vi "MDPtr GlobalSettings.vi"(6 "Oper(Get)":bool, 8 "error in (no error)":errorcluster, 11 "Setting in":T1) -> (0 "error out":errorcluster, 3 "Setting out":T1)   [LabVIEW 2017, in "MDPtr.lvlib"]
uses:
  MDPtr.lvlib
  MDPtr TypeDef/MDPtr GlobalSettings.ctl
  MDPtr TypeDef/MDPtr MallocMethod.ctl
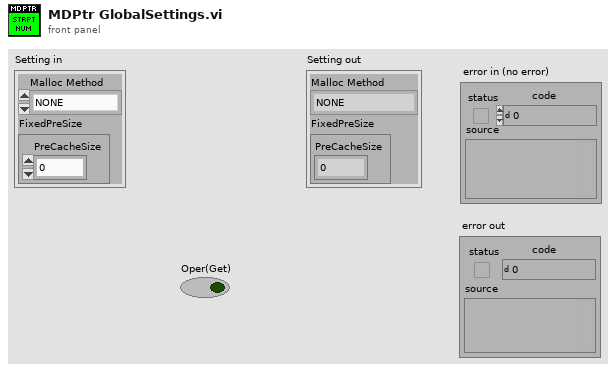
[diagram p1: front panel]
types:
  T1 = typedef "MDPtr.lvlib/MDPtr GlobalSettings.ctl" = cluster{"Malloc Method":T2, "FixedPreSize":cluster{"PreCacheSize":i32}}
  T2 = typedef "MDPtr.lvlib/MDPtr MallocMethod.ctl" = enum16{"NONE", "FIXED PRE-SIZE"}
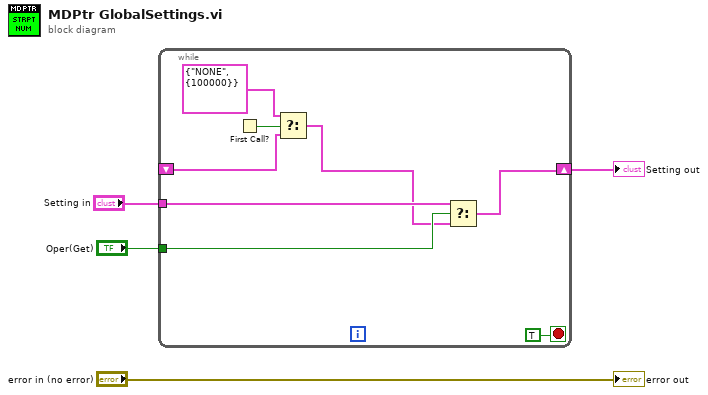
[diagram p0: block diagram]
diagram:
  n1 = while {
    tunnel: "Oper(Get)" -> [w10]
    shift-right: [w9] -> w3
    shift-left: _ -> [w6]
    tunnel: "Setting in" -> [w11]
    stop <- TRUE stop-if-true
    n2 = First Call?() -> (First Call?: T/F=w8:bool)
    n3 = Select(t=T1 {"Malloc Method"=enum."NONE", "FixedPreSize"={"PreCacheSize"=100000}} ("Cluster"), s=w8, f=w6) -> (s? t:f=w5:T1)
    n4 = Select(t=w11, s=w10, f=w5) -> (s? t:f=w9:T1)
  }
  "Setting out" <- w3
  "error out" <- "error in (no error)"
